vi "VIH - CHM Project - Get Actual HHP_Generation Params.vi"(11 "HHP_Generation":T1={"HHP_Template"=enum."default", "HHP_Template_CustomPath"=path "", "HHP_Target"=enum."default", "HHP_Target_CustomPath"=path "", "HHP_CreateTOC"=TRUE, "HHP_CreateIDX"=TRUE, "HHP_DefaultTopic"=enum."auto", "HHP_DefaultTopic_CustomPath"=path "", "CHM_Filename"=path "", "HHP_AutoBuild"=FALSE, "CHM_AutoBuild"=FALSE}) -> (0 "Abs CHM Path":bool, 1 "CHM File Absolute Path":path, 3 "HHP_Generation out":T1={"HHP_Template"=enum."default", "HHP_Template_CustomPath"=path "", "HHP_Target"=enum."default", "HHP_Target_CustomPath"=path "", "HHP_CreateTOC"=TRUE, "HHP_CreateIDX"=TRUE, "HHP_DefaultTopic"=enum."auto", "HHP_DefaultTopic_CustomPath"=path "", "CHM_Filename"=path "", "HHP_AutoBuild"=FALSE, "CHM_AutoBuild"=FALSE})   [LabVIEW 2014]
doc: "::: VI Helpeks :::\nCopyright (c) 2000-2026 Konstantin Shifershteyn. All rights reserved."
uses:
  VIH - CHM Project - HHP Generation Params Cluster.ctl
panel:
  # "VI Helpeks\nCopyright (c) 2012-2026 Konstantin Shifershteyn"
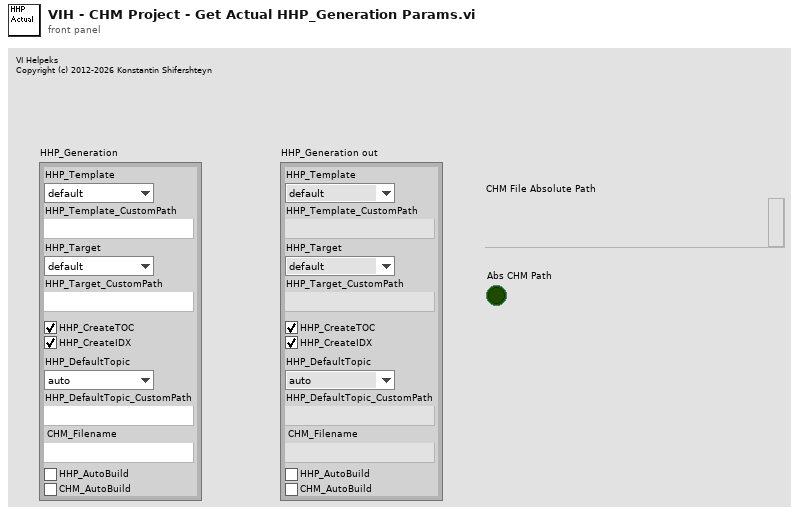
[diagram p1: front panel]
types:
  T1 = typedef "VIH - CHM Project - HHP Generation Params Cluster.ctl" = cluster{"HHP_Template":enum16{"default", "custom"}, "HHP_Template_CustomPath":path, "HHP_Target":enum16{"default", "custom"}, "HHP_Target_CustomPath":path, "HHP_CreateTOC":bool, "HHP_CreateIDX":bool, "HHP_DefaultTopic":enum16{"auto", "custom"}, "HHP_DefaultTopic_CustomPath":path, "CHM_Filename":path, "HHP_AutoBuild":bool, "CHM_AutoBuild":bool}
  T2 = typedef "VIH HelpGen Typedef - Cluster - Group Rule.ctl" = cluster{"Source Root Dir":path, "Build Root Dir":path, "BuildHelp":T3, "Source Paths":T4, "Target Paths":T5, "VIDscrMode":T6, "MenuDscrMode":T6, "MenuItemIcons":T3, "Control Rules":T7[], "Flags":T9, "Ctl_DscrMode":T6, "Ctl_ClustMembers":T3, "Ctl_EnumValues":T3, "%Comments":string, "PVIIDscrMode":T6, "VIDetailsMode":T6, "ProductInfoMode":T3, "ProductInfoText":string}
  T3 = typedef "VIH HelpGen Typedef - Enum - Default,Enable,Disable.ctl" = enum16{"Default", "Enable", "Disable"}
  T4 = typedef "VIH HelpGen Typedef - Cluster - Group Rule - Source Paths.ctl" = cluster{"CSS Files":path[], "JS Files":path[], "VI Template":path, "Menu Template":path, "PolyVI Template":path}
  T5 = typedef "VIH HelpGen Typedef - Cluster - Group Rule - Target Paths.ctl" = cluster{"HTML Dir":path, "Image Dir":path, "CSS Dir":path, "JS Dir":path}
  T6 = typedef "VIH HelpGen Typedef - Enum - Description Mode.ctl" = enum16{"Default", "Description", "Description1", "Description2", "Custom", "None"}
  T7 = typedef "VIH HelpGen Typedef - Cluster - Control Rule.ctl" = cluster{"CtrlID":string, "CustomRule":bool, "DscrMode":T6, "Description":string, "ClusterMembers":T3, "EnumValues":T3, "EnumValDscr":T8[], "CustomName":string}
  T8 = typedef "VIH HelpGen Typedef - Cluster - Enum Value Info.ctl" = cluster{"Value":ext, "String":string, "Description":string}
  T9 = typedef "VIH HelpGen Typedef - Cluster - Group Rule - Flags.ctl" = cluster{"Override CSS Files":bool, "Override JS Files":bool, "Override Ctl Rules":bool}
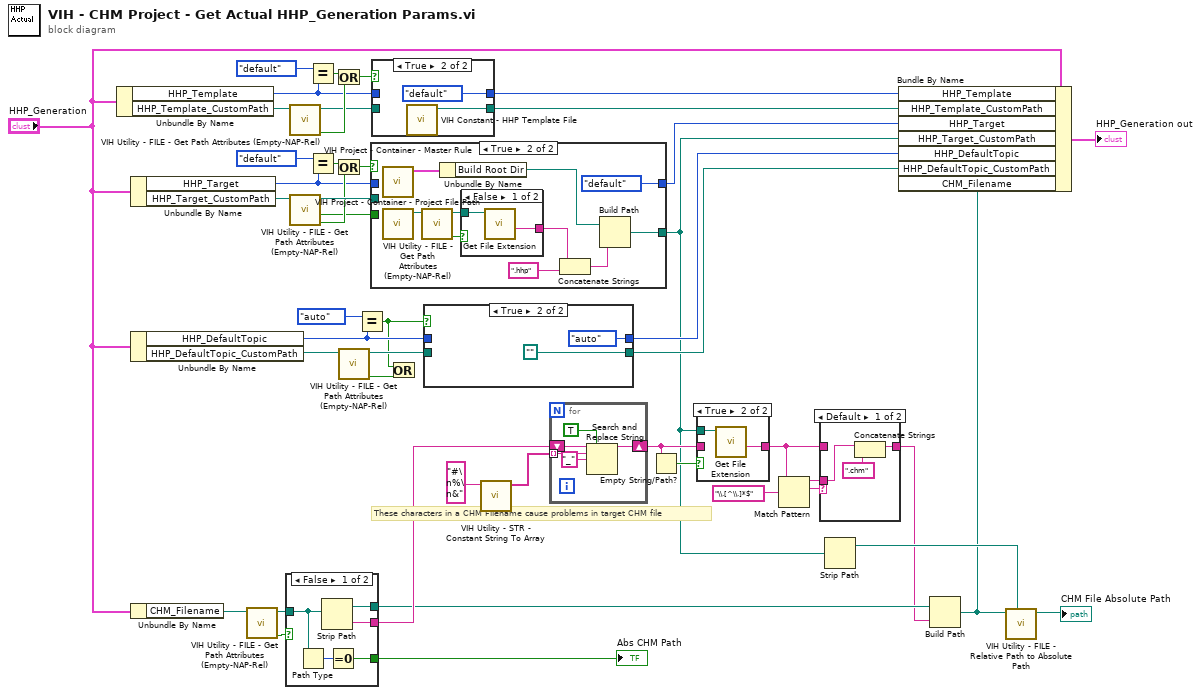
[diagram p0: block diagram]
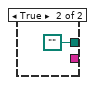
[diagram p2: hidden frame]
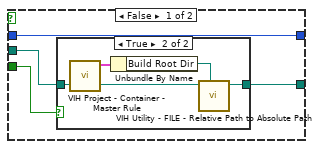
[diagram p6: hidden frame]
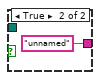
[diagram p8: hidden frame]
diagram:
  # "These characters in a CHM Filename cause problems in target CHM file"
  n1 = Unbundle By Name("HHP_Generation") -> ("HHP_Template"=w42:enum16{"default", "custom"}, "HHP_Template_CustomPath"=w46:path)
  n2 = Unbundle By Name("HHP_Generation") -> ("HHP_Target"=w32:enum16{"default", "custom"}, "HHP_Target_CustomPath"=w31:path)
  n3 = Unbundle By Name("HHP_Generation") -> ("HHP_DefaultTopic"=w26:enum16{"auto", "custom"}, "HHP_DefaultTopic_CustomPath"=w28:path)
  n4 = Unbundle By Name("HHP_Generation") -> ("CHM_Filename"=w2:path)
  n5 = call "VIH Utility - FILE - Get Path Attributes (Empty-NAP-Rel).vi"("Path"=w2) -> ("Not A Path or Empty path"=w11:bool, "dup Path"=w12:path)  [unwired: 6 in, 3 out]
  n6 = case shown="False" w11 {
    tunnel: w12 -> [w52 _]
    tunnel: [w51 _] -> w10
    tunnel: [w50 path "" ("stripped path")] -> w7
    tunnel: [w48 _] -> w4
    frame False {
      n7 = Path Type(1:w52) -> (0:w49:i16)
      n8 = Strip Path(path=w52) -> (stripped path=w50:path, name=w51:string)
      n9 = Equal To 0?(x=w49) -> (x = 0?=w48:bool)
    }
    frame True {
    }
  }
  "Abs CHM Path" <- w4
  n10 = call "VIH Utility - FILE - Get Path Attributes (Empty-NAP-Rel).vi"("Path"=w46) -> ("Not A Path or Empty path"=w45:bool, "dup Path"=w41:path)  [unwired: 6 in, 3 out]
  n11 = call "VIH Utility - FILE - Get Path Attributes (Empty-NAP-Rel).vi"("Path"=w31) -> ("Not A Path or Empty path"=w34:bool, "Relative path"=w1:bool, "dup Path"=w37:path)  [unwired: 6 in, 2 out]
  n12 = Equal?(x=enum16{"default", "custom"}."default", y=w42) -> (x = y?=w44:bool)
  n13 = Equal?(x=enum16{"default", "custom"}."default", y=w32) -> (x = y?=w35:bool)
  n14 = Or(x=w44, y=w45) -> (x .or. y?=w43:bool)
  n15 = Or(x=w35, y=w34) -> (x .or. y?=w36:bool)
  n16 = call "VIH Utility - FILE - Get Path Attributes (Empty-NAP-Rel).vi"("Path"=w28) -> ("Not A Path or Empty path"=w29:bool, "dup Path"=w25:path)  [unwired: 6 in, 3 out]
  n17 = Equal?(x=enum16{"auto", "custom"}."auto", y=w26) -> (x = y?=w16:bool)
  n18 = case shown="True" w36 {
    tunnel: [w57 enum16{"default", "custom"}."default" ("x")] -> w30
    tunnel: w32 -> [w57 _]
    tunnel: [w55 w66] -> w9
    tunnel: w37 -> [w54 _]
    tunnel: w1 -> [w56 _]
    frame False {
      n19 = case shown="True" w56 {
        tunnel: [w58 w60] -> w55
        tunnel: w54 -> [w58 w61]
        frame False {
        }
        frame True {
          n20 = call "VIH Project - Container - Master Rule.vi"() -> ("Rule out"=w62:T2)  [unwired: 11 in]
          n21 = Unbundle By Name(w62) -> ("Build Root Dir"=w59:path)
          n22 = call "VIH Utility - FILE - Relative Path to Absolute Path.vi"("base path (empty: dir of Top VI)"=w59, "Path"=w61) -> ("Path out"=w60:path)  [unwired: 8 in, 1 out]
        }
      }
    }
    frame True {
      n23 = call "VIH Project - Container - Master Rule.vi"() -> ("Rule out"=w67:T2)  [unwired: 11 in]
      n24 = call "VIH Project - Container - Project File Path.vi"() -> ("Project File Path"=w65:path)  [unwired: 9 in, 2 out]
      n25 = call "VIH Utility - FILE - Get Path Attributes (Empty-NAP-Rel).vi"("Path"=w65) -> ("Not A Path or Empty path"=w63:bool, "dup Path"=w64:path)  [unwired: 6 in, 3 out]
      n26 = Unbundle By Name(w67) -> ("Build Root Dir"=w70:path)
      n27 = case shown="False" w63 {
        tunnel: [w74 "unnamed" ("filename without extension")] -> w69
        tunnel: w64 -> [w73 _]
        frame False {
          n28 = call <vilib>:"Get File Extension.vi"("file"=w73) -> ("filename without extension"=w74:string)  [unwired: 7 in, 3 out]
        }
        frame True {
        }
      }
      n29 = Concatenate Strings(w69, ".hhp" ("string")) -> (w71:string)
      n30 = Build Path(base path=w70, name or relative path=w71) -> (appended path=w66:path)
    }
  }
  n31 = case shown="True" w43 {
    tunnel: [w77 enum16{"default", "custom"}."default" ("x")] -> w40
    tunnel: w42 -> [w77 _]
    tunnel: [w76 w78] -> w39
    tunnel: w41 -> [w76 _]
    frame False {
    }
    frame True {
      n32 = call "VIH Constant - HHP Template File.vi"() -> ("HHP Template File path"=w78:path)  [unwired: 11 in]
    }
  }
  n33 = Or(x=w16, y=w29) -> ()  [unwired: 1 out]
  n34 = case shown="True" w16 {
    tunnel: [w81 enum16{"auto", "custom"}."auto" ("HHP_DefaultTopic")] -> w24
    tunnel: w26 -> [w81 _]
    tunnel: [w80 path ""] -> w23
    tunnel: w25 -> [w80 _]
    frame False {
    }
    frame True {
    }
  }
  n35 = call "VIH Utility - STR - Constant String To Array.vi"("String in"="#\n%\n&") -> ("Array out"=w14:string[])  [unwired: 10 in]
  n36 = for {
    shift-right: [w86] -> w13
    shift-left: w10 -> [w88]
    tunnel: w14 -> [w85] mode=indexing
    n37 = Search and Replace String(replace all?=TRUE ("replace all? (F)"), input string=w88, search string=w85, replace string="_" ("replace string (\"\")")) -> (result string=w86:string)  [unwired: 4 in, 3 out]
  }
  n38 = Empty String/Path?(string/path=w13) -> (empty?=w21:bool)
  n39 = case shown="True" w21 {
    tunnel: w9 -> [_ w91]
    tunnel: [w89 w90] -> w20
    tunnel: w13 -> [w89 _]
    frame False {
    }
    frame True {
      n40 = call <vilib>:"Get File Extension.vi"("file"=w91) -> ("filename without extension"=w90:string)  [unwired: 7 in, 3 out]
    }
  }
  n41 = Match Pattern(string=w20, regular expression="\\.[^\\.]*$") -> (before substring=w17:string, match substring=w18:string)  [unwired: 1 in, 2 out]
  n42 = case shown="Default" w18 {
    tunnel: w20 -> [_ w95]
    tunnel: [w93 w95] -> w6
    tunnel: w17 -> [w92 _]
    frame Default {
      n43 = Concatenate Strings(w92, ".chm") -> (w93:string)
    }
    frame ".chm" {
    }
  }
  n44 = Strip Path(path=w9) -> (stripped path=w8:path)  [unwired: 1 out]
  n45 = Build Path(base path=w7, name or relative path=w6) -> (appended path=w3:path)
  n46 = Bundle By Name(cluster="HHP_Generation", "HHP_Template"=w40, "HHP_Template_CustomPath"=w39, "HHP_Target"=w30, "HHP_Target_CustomPath"=w9, "HHP_DefaultTopic"=w24, "HHP_DefaultTopic_CustomPath"=w23, "CHM_Filename"=w3) -> (→"HHP_Generation out":T1)
  n47 = call "VIH Utility - FILE - Relative Path to Absolute Path.vi"("base path (empty: dir of Top VI)"=w8, "Path"=w3) -> ("Path out"=→"CHM File Absolute Path":path)  [unwired: 8 in, 1 out]
